vi "GetLogFromErrorManager.vi"(8 "error in (no error)":errorcluster, 11 "CDependencyInspection in":refnum<class "CDependencyInspection.lvclass">) -> (0 "error out":errorcluster, 1 "Log results":string[][](array[string]), 3 "CDependencyInspection out":refnum<class "CDependencyInspection.lvclass">)   [LabVIEW 2020, in "DependencyInspection.lvlib" / "CDependencyInspection.lvclass"]
uses:
  CDependencyInspection.lvclass
  CDependencyInspection.lvclass/CDependencyInspection.ctl
  ErrorManager/ErrorManager/ErrorManager.lvclass
  ErrorManager/ErrorManager/ErrorType.ctl
  LabVIEWObjectInterfaces/IErrorManager/IErrorManager.lvclass
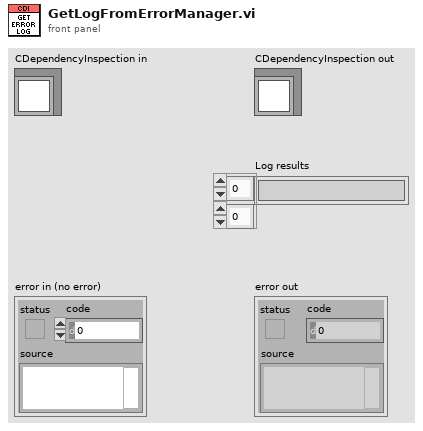
[diagram p1: front panel]
types:
  T1 = typedef "ErrorManager.lvlib/ErrorManager.lvclass/ErrorInfo.ctl" = cluster{"Time Stamp":timestamp, "Message":string, "Type":T2}
  T2 = typedef "LabVIEWObjectInterfaces.lvlib/IErrorManager.lvclass/ErrorType.ctl" = enum16{"Info", "Warning", "Error"}
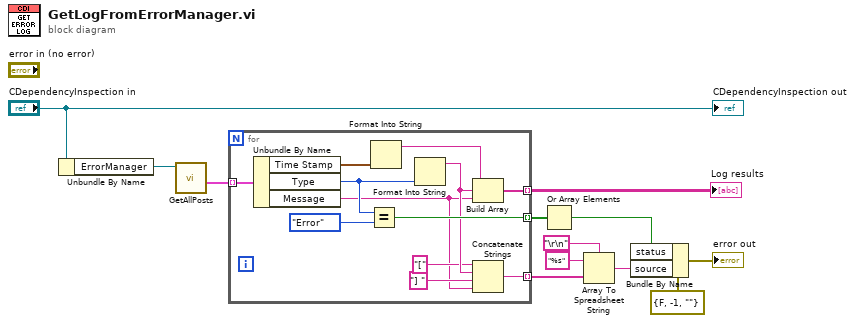
[diagram p0: block diagram]
diagram:
  n1 = Unbundle By Name("CDependencyInspection in") -> ("ErrorManager"=w11:refnum<class "ErrorManager.lvclass">)
  n2 = call-dynamic "GetAllPosts.vi"("ErrorManager in"=w11) -> ("Errors"=w10:T1[])  [unwired: 8 in, 2 out]
  n3 = for {
    tunnel: w10 -> [w24] mode=indexing
    tunnel: [w21] -> w9 mode=indexing
    tunnel: [w19] -> w8 mode=indexing
    tunnel: [w13] -> w5 mode=indexing
    n4 = Unbundle By Name(w24) -> ("Time Stamp"=w23:timestamp, "Type"=w18:T2, "Message"=w14:string)
    n5 = Equal?(x=w18, y=ErrorType."Error" ("Type")) -> (x = y?=w19:bool)
    n6 = Format Into String(w23) -> (resulting string=w22:string)  [unwired: 3 in, 1 out]
    n7 = Format Into String(w18) -> (resulting string=w17:string)  [unwired: 3 in, 1 out]
    n8 = Build Array(w22, w17, w14) -> (w21:string[])
    n9 = Concatenate Strings("[" ("string"), w17, "] " ("string"), w14) -> (w13:string)
  }
  "Log results" <- w9
  n10 = Or Array Elements(Boolean array=w8) -> (logical OR=w6:bool)
  n11 = Array To Spreadsheet String(delimiter (Tab)="\r\n", array=w5, 3:"%s" ("format string")) -> (spreadsheet string=w2:string)
  n12 = Bundle By Name(cluster=errorcluster {"status"=FALSE, "code"=-1, "source"=""} ("error out"), "status"=w6, "source"=w2) -> (→"error out":errorcluster)
  "CDependencyInspection out" <- "CDependencyInspection in"
